vi "Close.vi"(8 "error in (no error)":errorcluster, 11 "Client in":refnum<class "Client.lvclass">) -> (0 "error out":errorcluster)   [LabVIEW 2020, in "PV Access.lvlib" / "PVA Client.lvlib" / "Client.lvclass"]
doc: "Close the client."
uses:
  Client.lvclass
  PV Access.lvlib
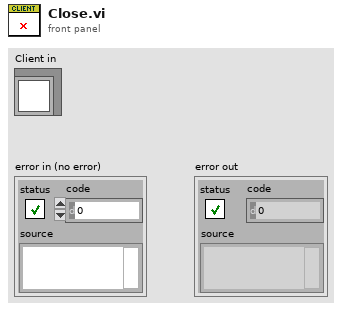
[diagram p1: front panel]
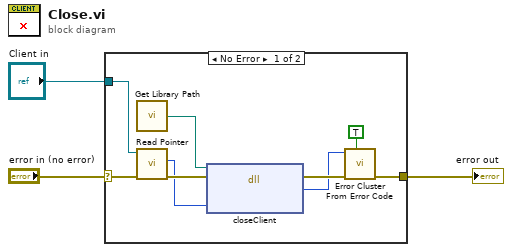
[diagram p0: block diagram]
diagram:
  n1 = case shown="No Error" "error in (no error)" {
    selector: "error in (no error)" -> [w8 w13]
    tunnel: [w11 w13] -> w2
    tunnel: "Client in" -> [w7 _]
    frame No Error {
      n2 = call "Get Library Path.vi"() -> ("Path"=w4:path)  [unwired: 1 in]
      n3 = call-dynamic "Read Pointer.vi"("error in (no error)"=w8, "Pointer Base in"=w7) -> ("error out"=w9:errorcluster, "Pointer"=w6:i64)  [unwired: 7 in, 1 out]
      n4 = dll-call lib="?" fn="closeClient"(path in=w4, error in=w9, "client"=w6) -> (error out=w12:errorcluster, "ret_code"=w10:i32)  [unwired: 2 in, 1 out]
      n5 = call <vilib>:"Error Cluster From Error Code.vi"("show call chain? (False)"=TRUE, "error in (no error)"=w12, "error code (0)"=w10) -> ("error out"=w11:errorcluster)  [unwired: 6 in]
    }
    frame Error {
    }
  }
  "error out" <- w2
